vi "MCLB_NameArray_Tests.vi"(11 "error in":errorcluster) -> (15 "error out":errorcluster)   [LabVIEW 2016, in "DronaTest.lvlib"]
uses:
  DronaTest.lvlib
  APIs/Stimulus/ControlValue/typedef/Name&Occurrence.ctl
  APIs/Stimulus/ControlValue/SetValueAuto.vi
  APIs/Stimulus/ControlValue/Controls/MC Listbox/SetValueByArrayName.vi
  APIs/Assert/AssertControlValue/Equal.vi
  APIs/Get/GetControlRef/GetControlRefByPath.vi
  <vilib>/addons/_JKI Toolkits/Caraya/classes/Test/Test.lvclass
  Drona.lvlib
  <vilib>/SLL Toolkit/SLL Debug/SLL Debug.lvlib
  APIs/Stimulus/ControlValue/ControlValue.lvlib
  APIs/Assert/AssertControlValue/AssertControlValue.lvlib
  <vilib>/addons/_JKI Toolkits/Caraya/classes/Assert/Assert.lvclass
  APIs/Stimulus/ControlValue/Controls/MC Listbox/StimulusMCListbox.lvlib
  APIs/Get/GetControlRef/GetControlRef.lvlib
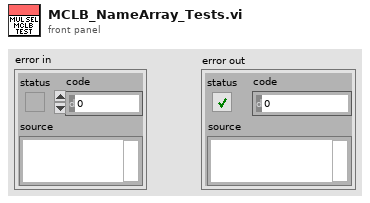
[diagram p1: front panel]
types:
  T1 = typedef "Drona.lvlib/ControlValue.lvlib/Name&Occurrence.ctl" = cluster{"ItemName":string, "Occurrence":i32}
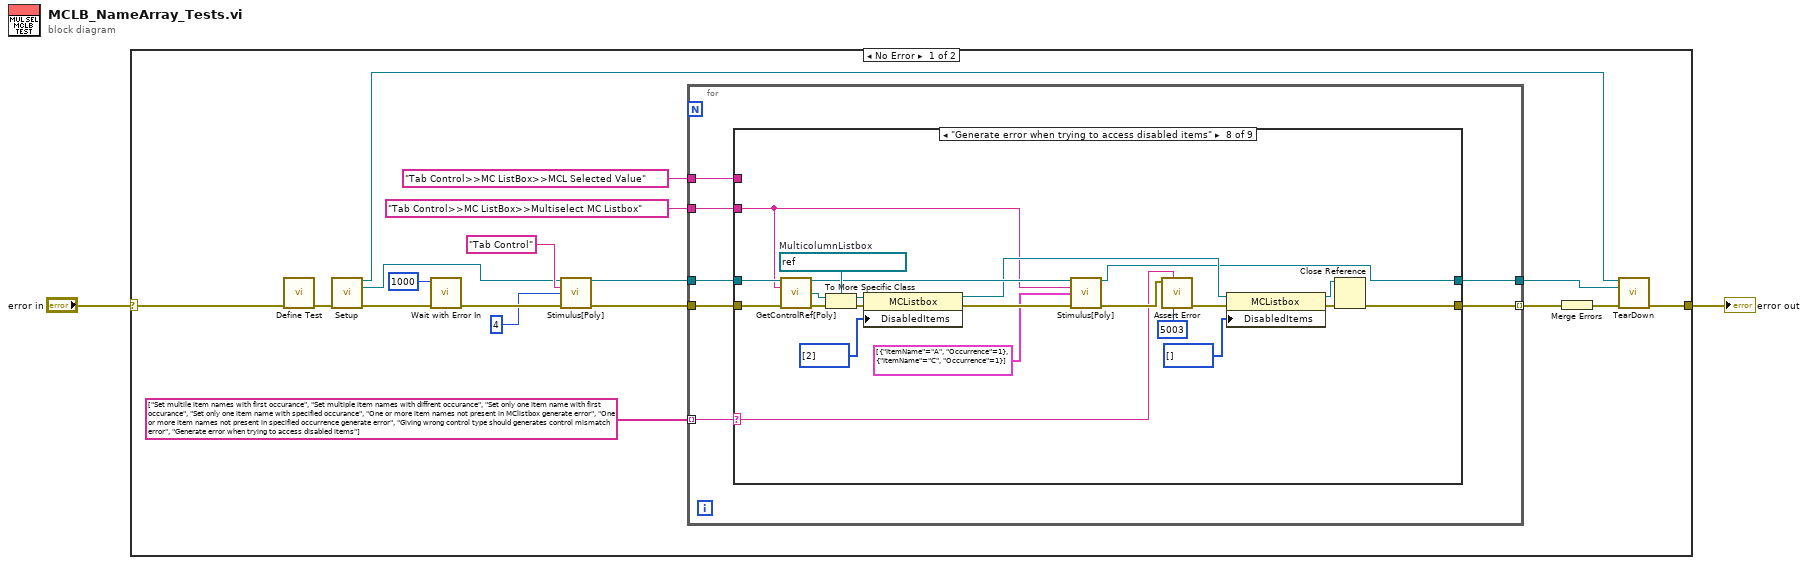
[diagram p0: block diagram]
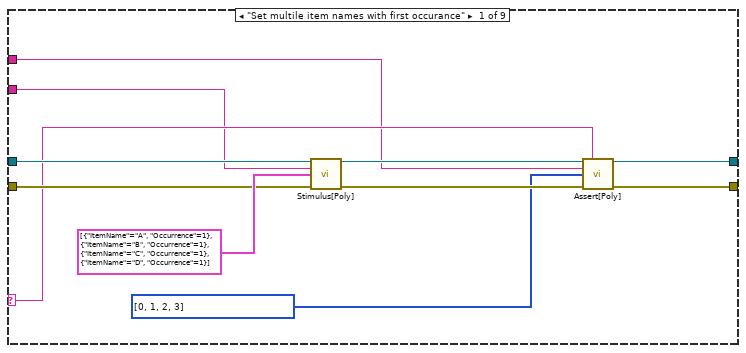
[diagram p2: hidden frame]
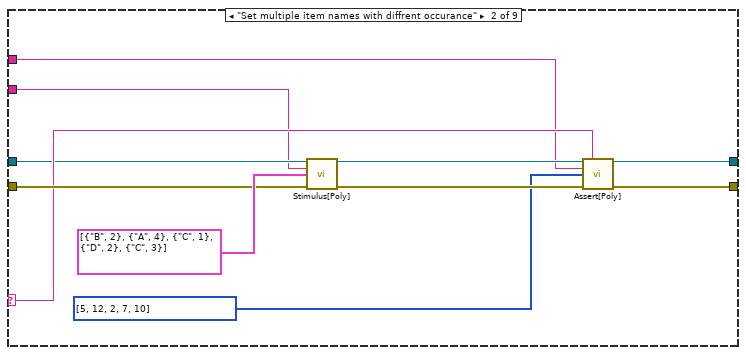
[diagram p3: hidden frame]
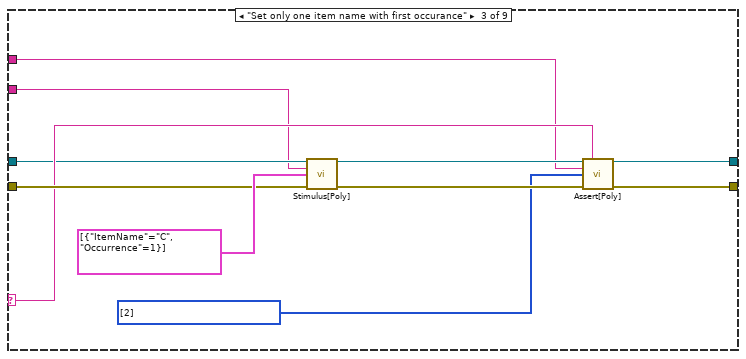
[diagram p4: hidden frame]
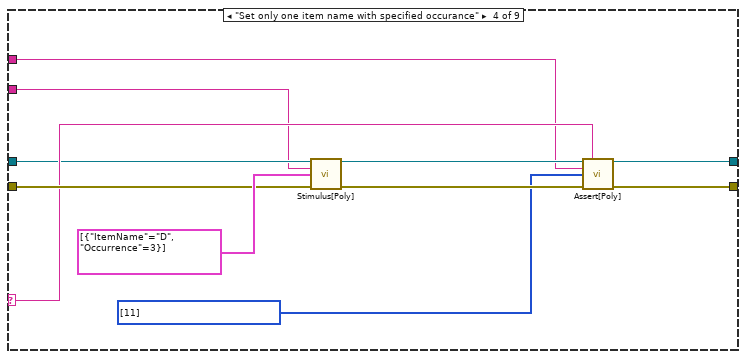
[diagram p5: hidden frame]
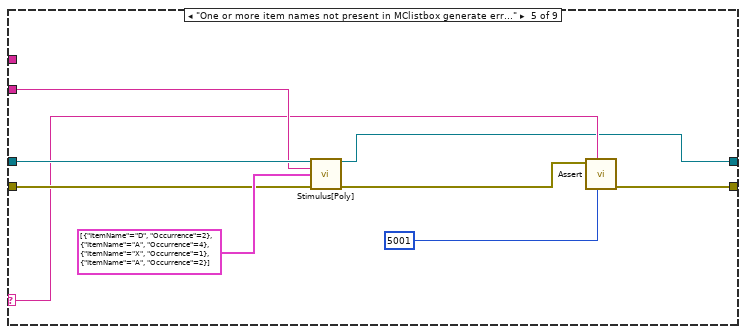
[diagram p6: hidden frame]
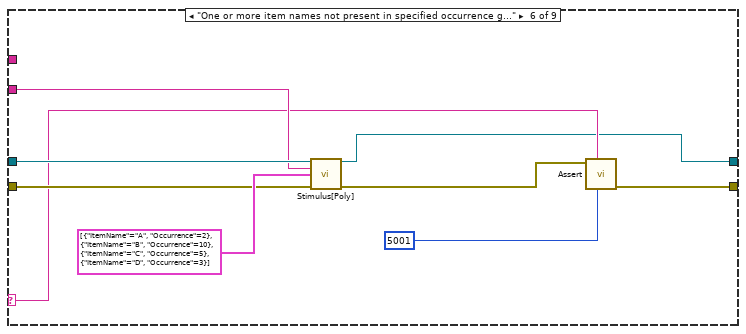
[diagram p7: hidden frame]
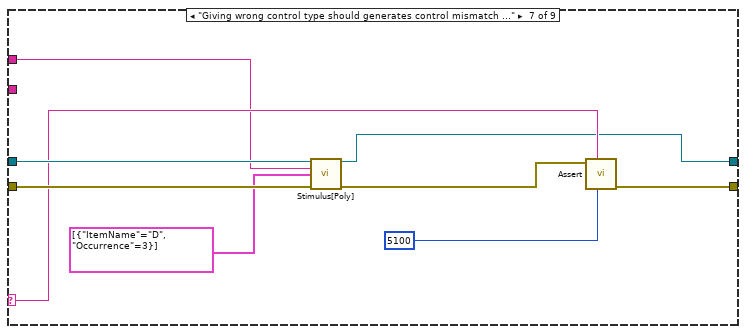
[diagram p8: hidden frame]
diagram:
  n1 = case shown="No Error" "error in" {
    selector: "error in" -> [w20 w123]
    tunnel: [w3 w123] -> w1
    frame No Error {
      n2 = call <vilib>:"Define Test.vi"("error in (no error)"=w20) -> ("error out"=w9:errorcluster)  [unwired: 9 in, 1 out]
      n3 = call "Setup.vi"("error in"=w9) -> ("Application Ref"=w4:refnum<vi>, "VI out"=w8:refnum<vi>, "error out"=w7:errorcluster)  [unwired: 12 in]
      n4 = call <vilib>:"Wait with Error In.vi"("error in (no error)"=w7, "milliseconds to wait"=u32 1000) -> ("error out"=w18:errorcluster)  [unwired: 9 in]
      n5 = call-poly "Stimulus[Poly].vi"("VI Reference In"=w8, "Control Path"="Tab Control", "Value (Signaling)"=4, "error in"=w18) -> ("VI Reference Out"=w14:refnum<vi>, "error out"=w13:errorcluster)  [unwired: 10 in]
      n6 = for {
        tunnel: [w27] -> w12 mode=indexing
        tunnel: [w26] -> w5
        tunnel: string[] ["Set multile item names with first occurance", "Set multiple item names with diffrent occurance", "Set only one item name with first occurance", "Set only one item name with specified occurance", "One or more item names not present in MClistbox generate error", "One or more item names not present in specified occurrence generate error", "Giving wrong control type should generates control mismatch error", "Generate error when trying to access disabled items"] -> [w25] mode=indexing
        tunnel: w14 -> [w24]
        tunnel: w13 -> [w23]
        tunnel: "Tab Control>>MC ListBox>>Multiselect MC Listbox" ("Control Path") -> [w22]
        tunnel: "Tab Control>>MC ListBox>>MCL Selected Value" ("Control Path") -> [w21]
        n7 = case shown="\"Generate error when trying to access disabled items\"" w25 {
          selector: w25 -> [w30 w42 w53 w64 w73 w82 w93 w101 _]
          tunnel: [w38 w49 w60 w71 w75 w84 w95 w103 w121] -> w27
          tunnel: [w37 w48 w59 w70 w72 w81 w92 w102 w122] -> w26
          tunnel: w24 -> [w31 w41 w52 w63 w78 w87 w97 w104 w122]
          tunnel: w23 -> [w32 w43 w54 w65 w79 w88 w98 w105 w121]
          tunnel: w22 -> [w28 w40 w51 w62 w77 w86 _ w99 _]
          tunnel: w21 -> [w29 w39 w50 w61 _ _ w90 _ _]
          frame "Set multile item names with first occurance" {
            n8 = call-poly "Stimulus[Poly].vi"("VI Reference In"=w31, "Control Path"=w28, "Name Array"=T1[] [{"ItemName"="A", "Occurrence"=1}, {"ItemName"="B", "Occurrence"=1}, {"ItemName"="C", "Occurrence"=1}, {"ItemName"="D", "Occurrence"=1}], "Error In"=w32) -> ("VI Reference Out"=w35:refnum<vi>, "Error Out"=w36:errorcluster)  [unwired: 10 in]
            n9 = call-poly "Assert[Poly].vi"("VI Reference In"=w35, "Test Label"=w30, "Control Path"=w29, "Control Value"=i32[] [0, 1, 2, 3] ("Index Array"), "Error In"=w36) -> ("VI Reference Out"=w37:refnum<vi>, "Error Out"=w38:errorcluster)  [unwired: 8 in, 1 out]
          }
          frame "Set multiple item names with diffrent occurance" {
            n10 = call-poly "Stimulus[Poly].vi"("VI Reference In"=w41, "Control Path"=w40, "Name Array"=T1[] [{"ItemName"="B", "Occurrence"=2}, {"ItemName"="A", "Occurrence"=4}, {"ItemName"="C", "Occurrence"=1}, {"ItemName"="D", "Occurrence"=2}, {"ItemName"="C", "Occurrence"=3}], "Error In"=w43) -> ("VI Reference Out"=w46:refnum<vi>, "Error Out"=w47:errorcluster)  [unwired: 10 in]
            n11 = call-poly "Assert[Poly].vi"("VI Reference In"=w46, "Test Label"=w42, "Control Path"=w39, "Control Value"=i32[] [5, 12, 2, 7, 10] ("Index Array"), "Error In"=w47) -> ("VI Reference Out"=w48:refnum<vi>, "Error Out"=w49:errorcluster)  [unwired: 8 in, 1 out]
          }
          frame "Set only one item name with first occurance" {
            n12 = call-poly "Stimulus[Poly].vi"("VI Reference In"=w52, "Control Path"=w51, "Name Array"=T1[] [{"ItemName"="C", "Occurrence"=1}], "Error In"=w54) -> ("VI Reference Out"=w57:refnum<vi>, "Error Out"=w58:errorcluster)  [unwired: 10 in]
            n13 = call-poly "Assert[Poly].vi"("VI Reference In"=w57, "Test Label"=w53, "Control Path"=w50, "Control Value"=i32[] [2] ("Index Array"), "Error In"=w58) -> ("VI Reference Out"=w59:refnum<vi>, "Error Out"=w60:errorcluster)  [unwired: 8 in, 1 out]
          }
          frame "Set only one item name with specified occurance" {
            n14 = call-poly "Stimulus[Poly].vi"("VI Reference In"=w63, "Control Path"=w62, "Name Array"=T1[] [{"ItemName"="D", "Occurrence"=3}], "Error In"=w65) -> ("VI Reference Out"=w68:refnum<vi>, "Error Out"=w69:errorcluster)  [unwired: 10 in]
            n15 = call-poly "Assert[Poly].vi"("VI Reference In"=w68, "Test Label"=w64, "Control Path"=w61, "Control Value"=i32[] [11] ("Index Array"), "Error In"=w69) -> ("VI Reference Out"=w70:refnum<vi>, "Error Out"=w71:errorcluster)  [unwired: 8 in, 1 out]
          }
          frame "One or more item names not present in MClistbox generate error" {
            n16 = call-poly "Stimulus[Poly].vi"("VI Reference In"=w78, "Control Path"=w77, "Name Array"=T1[] [{"ItemName"="D", "Occurrence"=2}, {"ItemName"="A", "Occurrence"=4}, {"ItemName"="X", "Occurrence"=1}, {"ItemName"="A", "Occurrence"=2}], "Error In"=w79) -> ("VI Reference Out"=w72:refnum<vi>, "Error Out"=w76:errorcluster)  [unwired: 10 in]
            n17 = call-poly <vilib>:"Assert.vi"("error code (1)"=5001, "Label"=w73, "Error?"=w76) -> ("error out"=w75:errorcluster)  [unwired: 7 in, 1 out]
          }
          frame "One or more item names not present in specified occurrence generate error" {
            n18 = call-poly "Stimulus[Poly].vi"("VI Reference In"=w87, "Control Path"=w86, "Name Array"=T1[] [{"ItemName"="A", "Occurrence"=2}, {"ItemName"="B", "Occurrence"=10}, {"ItemName"="C", "Occurrence"=5}, {"ItemName"="D", "Occurrence"=3}], "Error In"=w88) -> ("VI Reference Out"=w81:refnum<vi>, "Error Out"=w85:errorcluster)  [unwired: 10 in]
            n19 = call-poly <vilib>:"Assert.vi"("error code (1)"=5001, "Label"=w82, "Error?"=w85) -> ("error out"=w84:errorcluster)  [unwired: 7 in, 1 out]
          }
          frame "Giving wrong control type should generates control mismatch error" {
            n20 = call-poly "Stimulus[Poly].vi"("VI Reference In"=w97, "Control Path"=w90, "Name Array"=T1[] [{"ItemName"="D", "Occurrence"=3}], "Error In"=w98) -> ("VI Reference Out"=w92:refnum<vi>, "Error Out"=w96:errorcluster)  [unwired: 10 in]
            n21 = call-poly <vilib>:"Assert.vi"("error code (1)"=5100, "Label"=w93, "Error?"=w96) -> ("error out"=w95:errorcluster)  [unwired: 7 in, 1 out]
          }
          frame "Generate error when trying to access disabled items" {
            w117 = refnum<vi> refnum  # MulticolumnListbox
            n22 = call-poly "GetControlRef[Poly].vi"("VI Reference In"=w104, "Control Path"=w99, "error In"=w105) -> ("VI Reference Out"=w113:refnum<vi>, "Ctl Refnum"=w118:refnum<vi>, "error out"=w120:errorcluster)  [unwired: 10 in]
            n23 = To More Specific Class(target class=w117, reference=w118, error in=w120) -> (specific class reference=w116:refnum<vi>, error out=w119:errorcluster)
            n24 = property class="MCListbox"(reference=w116, error in=w119, "DisabledItems"=i32[] [2] ("Disabled Items")) -> (reference out=w111:refnum<vi>, error out=w114:errorcluster)
            n25 = call-poly "Stimulus[Poly].vi"("VI Reference In"=w113, "Control Path"=w99, "Name Array"=T1[] [{"ItemName"="A", "Occurrence"=1}, {"ItemName"="C", "Occurrence"=1}], "Error In"=w114) -> ("VI Reference Out"=w102:refnum<vi>, "Error Out"=w108:errorcluster)  [unwired: 10 in]
            n26 = call <vilib>:"Assert Error.vi"("error code (1)"=5003, "Label"=w101, "Error?"=w108) -> ("error out"=w107:errorcluster)  [unwired: 7 in, 1 out]
            n27 = property class="MCListbox"(reference=w111, error in=w107, "DisabledItems"=i32[] [] ("Disabled Items")) -> (reference out=w109:refnum<vi>, error out=w112:errorcluster)
            n28 = Close Reference(reference=w109, error in (no error)=w112) -> (error out=w103:errorcluster)
          }
          frame Default {
          }
        }
      }
      n29 = Merge Errors(w12) -> (w6:errorcluster)
      n30 = call "TearDown.vi"("Application Ref"=w4, "VI in"=w5, "error in (no error)"=w6) -> ("error out"=w3:errorcluster)  [unwired: 12 in]
    }
    frame Error {
    }
  }
  "error out" <- w1
